vi "findEdge.vi"(0 "reference":refnum<class "Graph.lvclass">, 1 "point2D":T1 {"y" format="%.2f"; "x" format="%.2f"}, 2 "GraphicsRef":refnum<class "Graphics.lvclass">, 5 "error in (no error)":errorcluster) -> (14 "reference out":refnum<class "Graph.lvclass">, 15 "edge":refnum<class "AbstractEdge.lvclass">, 16 "found":bool, 19 "error out":errorcluster)   [LabVIEW 2020, in "Graph.lvclass"]
uses:
  <resource>/Framework/Providers/Open_GDS/UML/Graph_class/Graph.lvclass
  <resource>/Framework/Providers/Open_GDS/UML/General/Point/Point Point2D.ctl
  <resource>/Framework/Providers/Open_GDS/UML/AbstractEdge_class/AbstractEdge.lvclass
  <resource>/Framework/Providers/Open_GDS/UML/Graphics_class/Graphics.lvclass
  <resource>/Framework/Providers/Open_GDS/UML/GeneralPathEdge_class/GeneralPathEdge.lvclass
  C:/Program Files (x86)/National Instruments/LabVIEW 2020/resource/Framework/Providers/Open_GDS/UML/AbstractEdge_class/AbstractEdge.lvclass
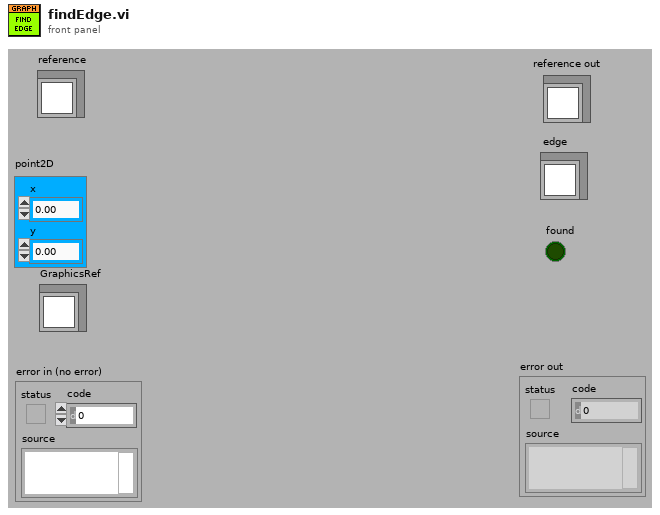
[diagram p1: front panel]
types:
  T1 = typedef "Point Point2D.ctl" = cluster{"x":dbl, "y":dbl}
  T2 = typedef "Graph.lvclass/ObjectAttributes.ctl" = cluster{"nodes":refnum<class "AbstractNode.lvclass">[], "edges":refnum<class "AbstractEdge.lvclass">[], "nodesToBeRemoved":refnum<class "AbstractNode.lvclass">[], "edgesToBeRemoved":refnum<class "AbstractEdge.lvclass">[], "needsLayout":bool, "LayoutNodes":refnum<class "AbstractNode.lvclass">[]}
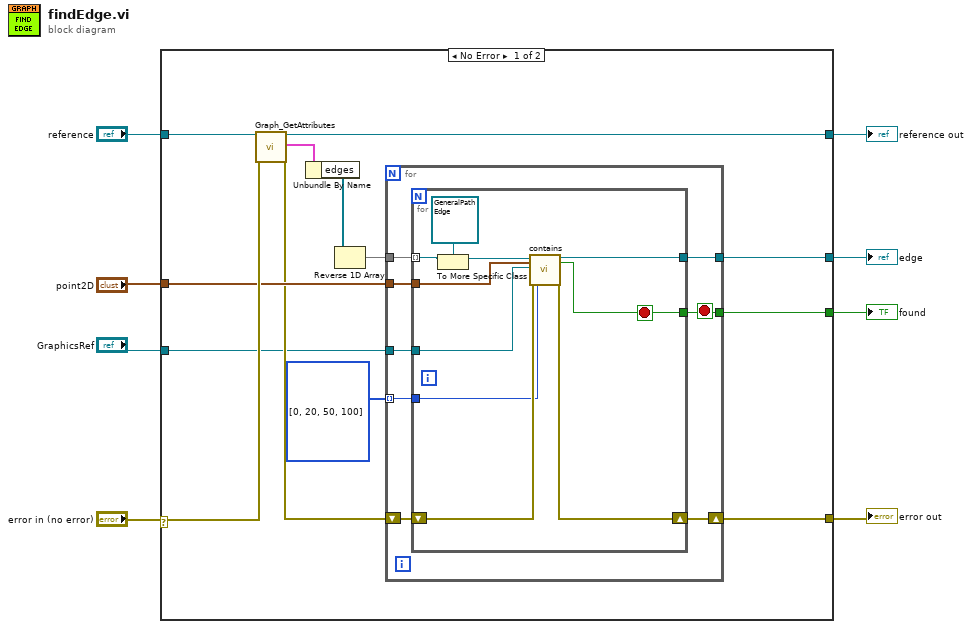
[diagram p0: block diagram]
diagram:
  n1 = case shown="No Error" "error in (no error)" {
    selector: "error in (no error)" -> [w18 w40]
    tunnel: "reference" -> [w21 w41]
    tunnel: [w20 w40] -> w7
    tunnel: [w19 w41] -> w6
    tunnel: "point2D" -> [w17 _]
    tunnel: [w16 _] -> w3
    tunnel: [w15 _] -> w2
    tunnel: "GraphicsRef" -> [w12 _]
    frame No Error {
      n2 = call <resource>:"Graph_GetAttributes.vi"("reference in"=w21, "error in (no error)"=w18) -> ("reference out"=w19:refnum<class "Graph.lvclass">, "Data"=w11:T2, "error out"=w13:errorcluster)  [unwired: 1 in, 14 out]
      n3 = Unbundle By Name(w11) -> ("edges"=w14:refnum<class "AbstractEdge.lvclass">[])
      n4 = Reverse 1D Array(array=w14) -> (reversed array=w10:refnum<class "AbstractEdge.lvclass">[])
      n5 = for {
        tunnel: w17 -> [w28]
        tunnel: [w27] -> w16
        tunnel: [w23] -> w15
        tunnel: w12 -> [w25]
        tunnel: w10 -> [w24]
        shift-right: [w29] -> w20
        shift-left: w13 -> [w26]
        tunnel: i32[] [0, 20, 50, 100] ("DistanceAwayOffset(100%)") -> [w22] mode=indexing
        stop <- w23 stop-if-true
        n6 = for {
          tunnel: w24 -> [w33] mode=indexing
          shift-right: [w38] -> w29
          shift-left: w26 -> [w39]
          tunnel: [w37] -> w27
          tunnel: w28 -> [w36]
          tunnel: [w31] -> w23
          tunnel: w25 -> [w32]
          tunnel: w22 -> [w30]
          stop <- w31 stop-if-true
          n7 = To More Specific Class(target class=refnum<class "GeneralPathEdge.lvclass"> refnum ("reference out"), reference=w33) -> (specific class reference=w35:refnum<class "GeneralPathEdge.lvclass">)  [unwired: 1 in, 1 out]
          n8 = call-dynamic "contains.vi"("reference"=w35, "point2D"=w36, "GraphicsRef"=w32, "error in (no error)"=w39, "DistanceAwayOffset(100%)"=w30) -> ("reference out"=w37:refnum<class "GeneralPathEdge.lvclass">, "contains"=w31:bool, "error out"=w38:errorcluster)  [unwired: 12 in]
        }
      }
    }
    frame Error {
    }
  }
  "reference out" <- w6
  "error out" <- w7
  "found" <- w2
  "edge" <- w3
